vi "Convert I2C Data & Buffer.vi"(5 "Status Ref":refnum<vi>, 8 "error in (no error)":errorcluster, 11 "Data":u8[](array[numeric])) -> (0 "error out":errorcluster)   [LabVIEW 2025, in "I2C Bus Monitor UI.lvlib"]
uses:
  I2C Bus Monitor UI.lvlib
  Table Buffer - Enqueue.vi
  Error Global.vi
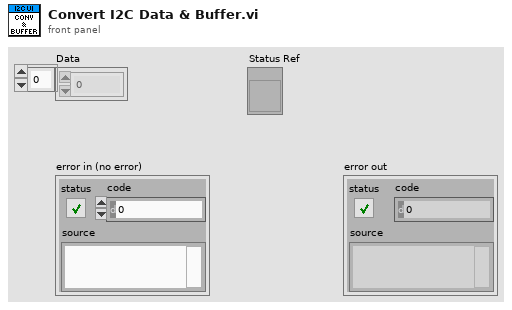
[diagram p1: front panel]
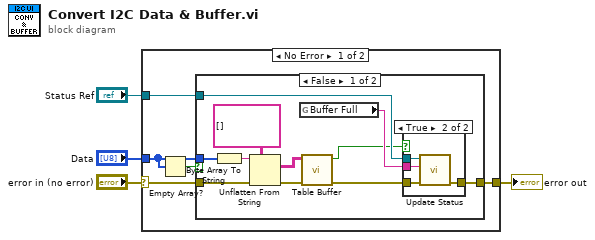
[diagram p0: block diagram]
diagram:
  n1 = case shown="No Error" "error in (no error)" {
    selector: "error in (no error)" -> [w6 w27]
    tunnel: [w9 w27] -> w4
    tunnel: "Data" -> [w8 _]
    tunnel: "Status Ref" -> [w5 _]
    frame No Error {
      n2 = Empty Array?(array=w8) -> (empty?=w7:bool)
      n3 = case shown="False" w7 {
        tunnel: w6 -> [w16 w26]
        tunnel: w8 -> [w18 _]
        tunnel: [w10 w26] -> w9
        tunnel: w5 -> [w13 _]
        frame False {
          n4 = Byte Array To String(unsigned byte array=w18) -> (string=w19:string)
          n5 = Unflatten From String(type=string[][] [] ("Fetched I2C Messages"), binary string=w19, error in (no error)=w16) -> (value=w15:string[][], error out=w17:errorcluster)  [unwired: 2 in, 1 out]
          n6 = global read "Error Global.vi" "Buffer Full"() -> (w14:string)
          n7 = call-poly "Table Buffer.vi"("error in (no error)"=w17, "Data"=w15) -> ("error out"=w12:errorcluster, "Overflow"=w11:bool)  [unwired: 8 in]
          n8 = case shown="True" w11 {
            tunnel: w12 -> [w21 w25]
            tunnel: w13 -> [_ w24]
            tunnel: [w21 w23] -> w10
            tunnel: w14 -> [_ w22]
            frame False {
            }
            frame True {
              n9 = call "Update Status.vi"("error in (no error)"=w25, "Value"=w22, "Status Ref"=w24) -> ("error out"=w23:errorcluster)  [unwired: 8 in]
            }
          }
        }
        frame True {
        }
      }
    }
    frame Error {
    }
  }
  "error out" <- w4
